vi "Center Dialog on Caller.vi"(8 "error in":errorcluster, 9 "Dialog VI":refnum<vi>, 11 "Calling VI in":refnum<vi>) -> (0 "error out":errorcluster)   [LabVIEW 2020]
doc: "Centers the front panel of a dialog VI in relation to the calling VI."
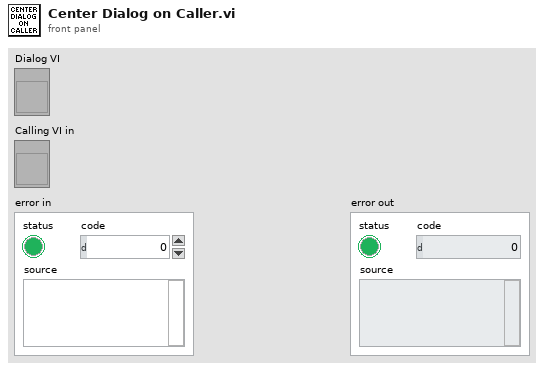
[diagram p1: front panel]
types:
  T1 = typedef "LVAllMonitorsDisplayTypeDef.ctl" = cluster{"Bounds":cluster{"Left":i16, "Top":i16, "Right":i16, "Bottom":i16}, "Depth":i16}[]
  T2 = typedef "LVRectTypeDef.ctl" = cluster{"Left":i16, "Top":i16, "Right":i16, "Bottom":i16}
  T3 = cluster{"left":i16, "top":i16, "right":i16, "bottom":i16}
  T4 = cluster{"Bounds":cluster{"Left":i16, "Top":i16, "Right":i16, "Bottom":i16}, "Depth":i16}
  T5 = cluster{"Left":i16, "Top":i16, "Right":i16, "Bottom":i16}
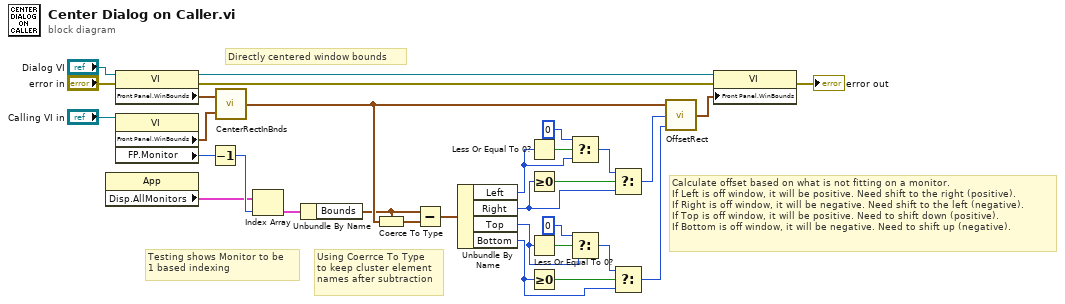
[diagram p0: block diagram]
diagram:
  # "Testing shows Monitor to be\n1 based indexing"
  # "Directly centered window bounds"
  # "Calculate offset based on what is not fitting on a monitor.\nIf Left is off window, it will be positive. Need shift to the right (positive).\nIf Right is off window, it will be negative. Need shift to the left (negative).\nIf Top is off window, it will be positive. Need to shift down (positive).\nIf Bottom is off window, it will be negative. Need to shift up (negative)."
  # "Using Coerrce To Type\nto keep cluster element\nnames after subtraction"
  n1 = property class="App"() -> ("Disp.AllMonitors"=w9:T1)  [unwired: 2 in, 2 out]
  n2 = property class="VI"(reference="Dialog VI", error in="error in") -> (reference out=w4:refnum<vi>, error out=w31:errorcluster, "Front Panel.WinBounds"=w6:T2)
  n3 = property class="VI"(reference="Calling VI in") -> ("Front Panel.WinBounds"=w2:T2, "FP.Monitor"=w7:u16)  [unwired: 1 in, 2 out]
  n4 = Decrement(x=w7) -> (x-1=w10:u16)
  n5 = call <vilib>:"CenterRectInBnds.vi"("bounds"=w2, "rect"=w6) -> ("centered rect"=w28:T3)
  n6 = Index Array(array=w9, index=w10) -> (element=w8:T4)
  n7 = Unbundle By Name(w8) -> ("Bounds"=w12:T5)
  n8 = Coerce To Type(0:w28, 1:w12) -> (2:w11:T5)
  n9 = Subtract(x=w12, y=w11) -> (x-y=w13:T5)
  n10 = Unbundle By Name(w13) -> ("Left"=w1:i16, "Right"=w18:i16, "Top"=w23:i16, "Bottom"=w24:i16)
  n11 = Less Or Equal To 0?(x=w1) -> (x <= 0?=w14:bool)
  n12 = Greater Or Equal To 0?(x=w18) -> (x >= 0?=w16:bool)
  n13 = Less Or Equal To 0?(x=w23) -> (x <= 0?=w22:bool)
  n14 = Greater Or Equal To 0?(x=w24) -> (x >= 0?=w20:bool)
  n15 = Select(t=i16 0 ("Left"), s=w14, f=w1) -> (s? t:f=w17:i16)
  n16 = Select(t=i16 0 ("Left"), s=w22, f=w23) -> (s? t:f=w19:i16)
  n17 = Select(t=w17, s=w16, f=w18) -> (s? t:f=w26:i16)
  n18 = Select(t=w19, s=w20, f=w24) -> (s? t:f=w27:i16)
  n19 = call <vilib>:"OffsetRect.vi"("v"=w27, "h"=w26, "rect"=w28) -> ("offset rect"=w25:T3)
  n20 = property class="VI"(reference=w4, error in=w31, "Front Panel.WinBounds"=w25) -> (error out=→"error out":errorcluster)  [unwired: 1 out]
